vi "conveyor to conveyor.vi"(2 "error in (no error)":errorcluster) -> (0 "error out":errorcluster)   [LabVIEW 2019]
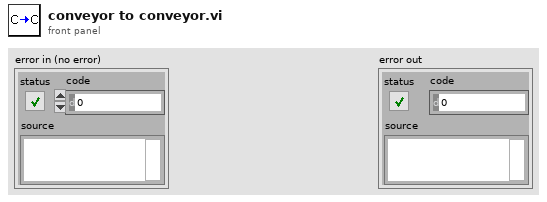
[diagram p1: front panel]
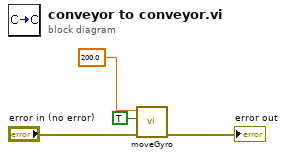
[diagram p0: block diagram]
diagram:
  n1 = call "moveGyro.vi"("error in (no error)"="error in (no error)", "タは"=TRUE, "移動距離"=200.0) -> ("error out"=→"error out":errorcluster)  [unwired: 8 in]
